vi "test1-testModuleExitEventAPI.vi"(8 "error in (no error)":errorcluster, 11 "TestCase in":refnum<class "testcase-CSMNonCSMCallerSupportAPI.lvclass">) -> (0 "error out":errorcluster, 3 "TestCase out":refnum<class "testcase-CSMNonCSMCallerSupportAPI.lvclass">)   [LabVIEW 2017, in "testcase-CSMNonCSMCallerSupportAPI.lvclass"]
uses:
  testcase-CSMNonCSMCallerSupportAPI.lvclass
  InternalCluster.ctl
  State_Cluster.ctl
  GlobalVariable_CSMModeData.vi
  <vilib>/addons/_JKI Toolkits/VI Tester/TestCase.llb/TestCase.lvclass
  src/user.lib/_NEVSTOP/Communicable State Machine(CSM)/Communicable State Machine.lvlib
  C:/Program Files (x86)/National Instruments/LabVIEW 2017/vi.lib/addons/_JKI Toolkits/VI Tester/TestCase.llb/TestCase.lvclass
panel:
  out "LoopCount":i32
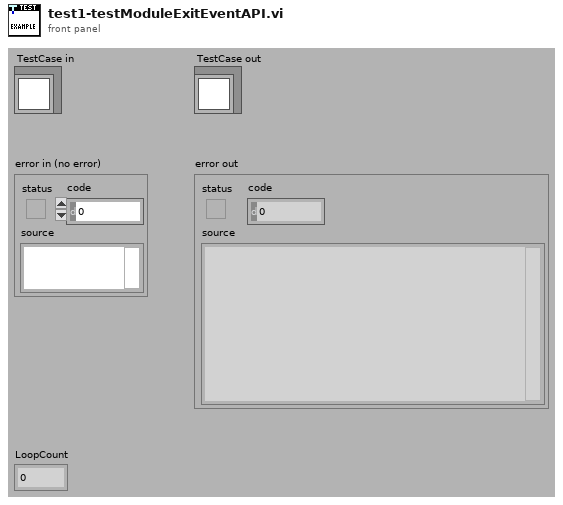
[diagram p1: front panel]
types:
  T1 = typedef "testcase-CSMNonCSMCallerSupportAPI.lvclass/InternalCluster.ctl" = cluster{"Mode":enum16{"Invalid", "Others", "WorkerAgent or Chain"}, "#Nodes":u32}
  T2 = typedef "testcase-CSMNonCSMCallerSupportAPI.lvclass/State_Cluster.ctl" = enum16{"Idle", "Initialize", "PreExit", "Exit"}
  T3 = enum16{"Invalid", "Others", "WorkerAgent or Chain"}
  T4 = typedef "Communicable State Machine.lvlib/_CSM_MODE.ctl" = enum16{"Not Exist", "Stand Alone", "CSM", "Worker", "Worker Agent", "Chain Node", "Chain"}
  T5 = cluster{"Module Exit event occured":bool, "Exit until all nodes exited":bool}
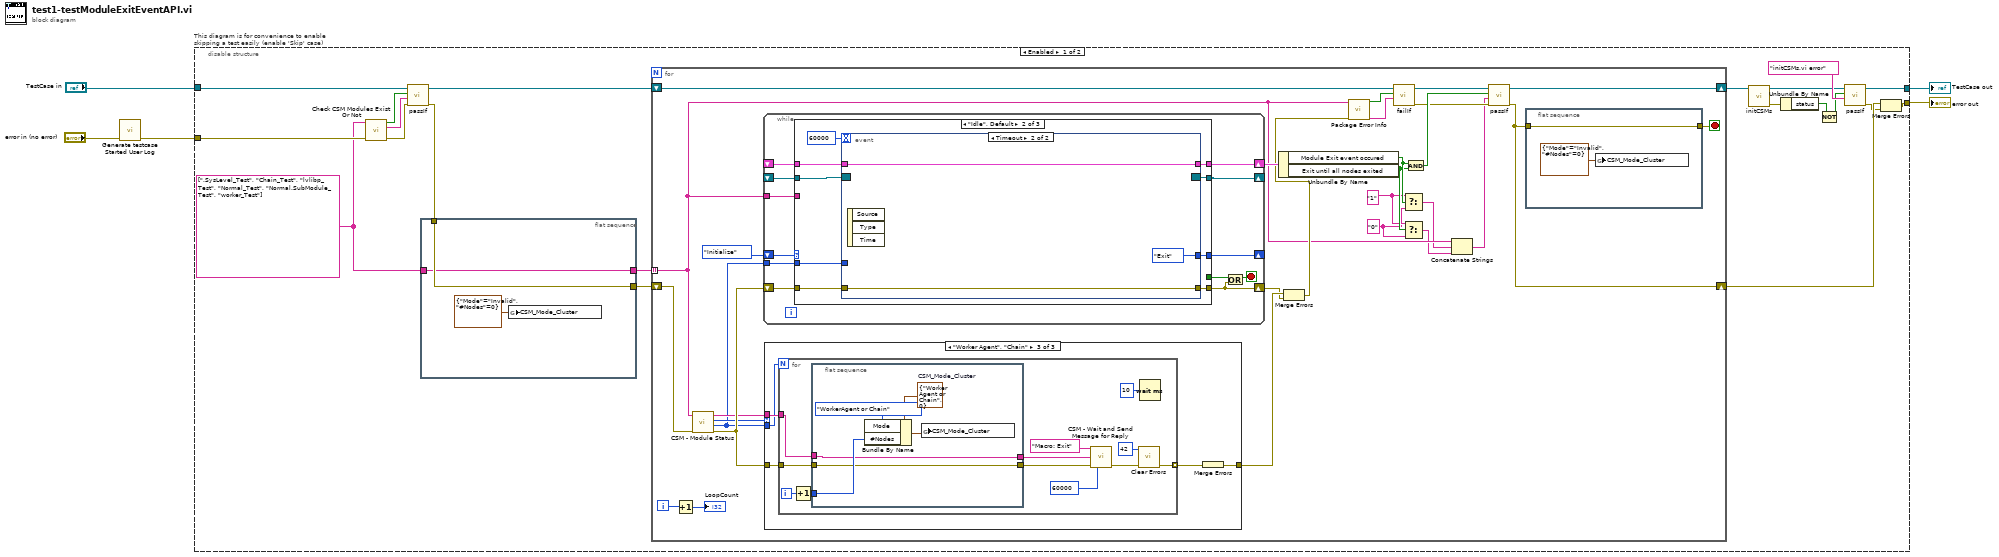
[diagram p0: block diagram]
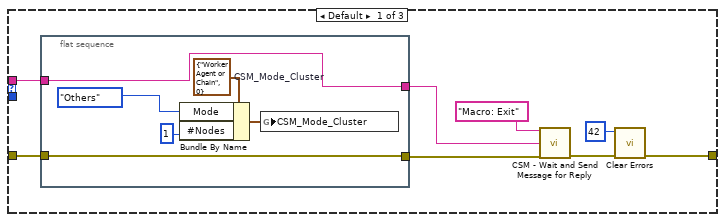
[diagram p2: hidden frame]
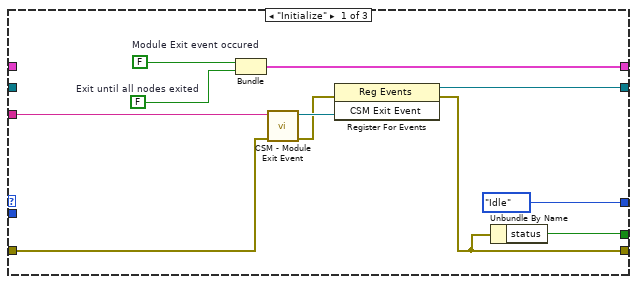
[diagram p4: hidden frame]
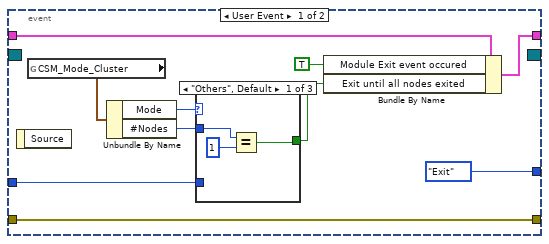
[diagram p5: hidden frame]
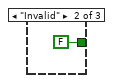
[diagram p6: hidden frame]
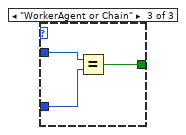
[diagram p7: hidden frame]
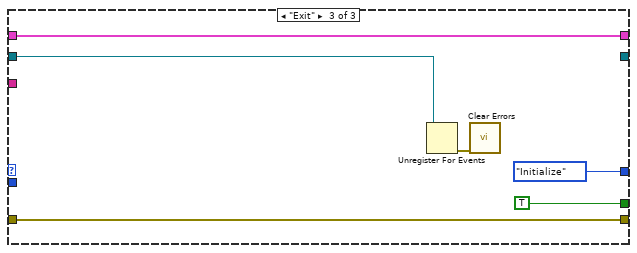
[diagram p8: hidden frame]
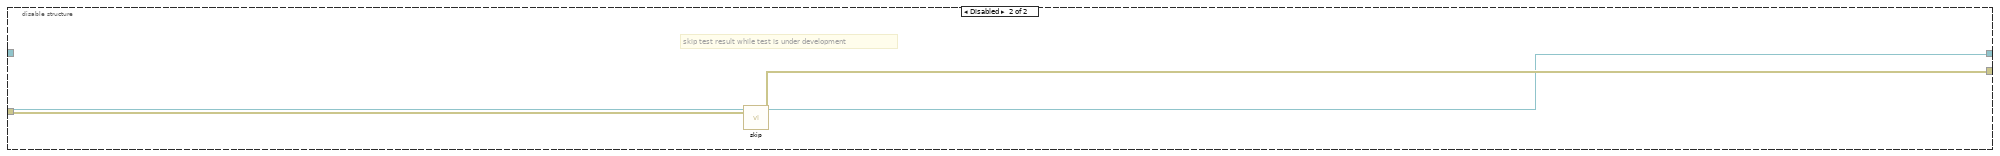
[diagram p9: hidden frame]
diagram:
  n1 = call "Generate testcase Started User Log.vi"("Error In"="error in (no error)") -> ("error out"=w1:errorcluster)  [unwired: 10 in]
  n2 = disable-structure "This diagram is for convenience to enable skipping a test easily (enable 'Skip' case)" shown="Enabled" {
    disable-tunnel: "TestCase in" -> [w18 w159]
    disable-tunnel: [w8 w157] -> w2
    disable-tunnel: [w23 w158] -> w4
    disable-tunnel: w1 -> [w16 w156]
    frame Enabled {
      w6 = string[] [".SysLevel_Test", "Chain_Test", "lvlibp_Test", "Normal_Test", "Normal.SubModule_Test", "worker_Test"] ("Module Names in All Scope")
      n3 = call "Check CSM Modules Exist Or Not.vi"("error in"=w16, "CSM names in"=w6) -> ("error out"=w19:errorcluster, "Debug string"=w20:string, "All Modules Exist?"=w21:bool)  [unwired: 7 in]
      n4 = call-dynamic "passIf.vi"("error in (no error)"=w19, "message (\"\")"=w20, "pass"=w21, "TestCase in"=w18) -> ("error out"=w15:errorcluster, "TestCase out"=w17:refnum<class "testcase-CSMNonCSMCallerSupportAPI.lvclass">)  [unwired: 6 in]
      n5 = flat-sequence {
        tunnel: [w27] -> w25
        tunnel: [w26] -> w22
        tunnel: w15 -> [w27]
        tunnel: w6 -> [w26]
        frame #0 {
          n6 = global write "GlobalVariable_CSMModeData.vi" "CSM_Mode_Cluster"(T1 {"Mode"=enum."Invalid", "#Nodes"=0} ("CSM_Mode_Cluster")) -> ()
        }
      }
      n7 = for {
        shift-right: [w38] -> w14
        shift-left: w25 -> [w52]
        shift-right: [w45] -> w24
        shift-left: w17 -> [w42]
        tunnel: w22 -> [w33] mode=indexing
        i -> [w56]
        stop <- w46 stop-if-true
        w34 = "0"
        w35 = "1"
        n8 = Increment(x=w56) -> (x+1=→"LoopCount":i32)
        n9 = call "CSM - Module Status.vi"("Error In"=w52, "CSM Name"=w33) -> ("error out"=w50:errorcluster, "#Nodes"=w47:i32, "Mode"=w49:T4, "CSM Name (Dup)"=w48:string)  [unwired: 5 in, 1 out]
        n10 = while {
          shift-right: [w105] -> _
          shift-left: State_Cluster."Initialize" -> [w103]
          shift-right: [w108] -> _
          shift-left: _ -> [w107]
          shift-right: [w106] -> w54
          shift-left: _ -> [w104]
          shift-right: [w98] -> w29
          shift-left: w50 -> [w101]
          tunnel: w47 -> [w102]
          tunnel: w33 -> [w100]
          stop <- w99 stop-if-true
          n11 = case shown="\"Idle\", Default" w103 {
            tunnel: [w117 _ TRUE] -> w109
            tunnel: [w119 w128 _] -> w108
            tunnel: w107 -> [_ w129 w155]
            tunnel: [w112 w126 w153] -> w106
            tunnel: w104 -> [_ w127 w153]
            tunnel: w101 -> [w118 w123 w151]
            tunnel: [w115 w122 w151] -> w98
            tunnel: [State_Cluster."Idle" w124 State_Cluster."Initialize"] -> w105
            tunnel: w102 -> [_ w121 _]
            tunnel: w100 -> [w110 _ _]
            frame "Initialize" {
              w111 = FALSE  # Exit until all nodes exited
              w113 = FALSE  # Module Exit event occured
              n12 = Bundle("Module Exit event occured"=w113, "Exit until all nodes exited"=w111) -> (w112:T5)  [unwired: 1 in]
              n13 = call "CSM - Module Exit Event.vi"("Error In"=w118, "Name (\"\" to Use UUID) In"=w110) -> ("error out"=w116:errorcluster, "CSM Exit Event"=w120:refnum<user-event>)  [unwired: 7 in, 1 out]
              n14 = register-events(error in=w116, w120) -> (reference out=w119:refnum<event-registration>, error out=w115:errorcluster)  [unwired: 1 in]
              n15 = Unbundle By Name(w115) -> ("status"=w117:bool)
            }
            frame "Idle", Default {
              n16 = event shown="[1] Timeout" {
                selector: w129 -> [_ _]
                dyn-events: [_ _] -> w128
                timeout: 60000 -> [_ _]
                tunnel: [State_Cluster."Exit" State_Cluster."Exit"] -> w124
                tunnel: w127 -> [w138 w149]
                tunnel: [w131 w149] -> w126
                tunnel: w123 -> [w136 w147]
                tunnel: [w136 w147] -> w122
                tunnel: w121 -> [w132 _]
                event User Event {
                  n17 = event-data() -> ()  [unwired: 1 in, 1 out]
                  n18 = global read "GlobalVariable_CSMModeData.vi" "CSM_Mode_Cluster"() -> (w135:T1)
                  n19 = Unbundle By Name(w135) -> ("Mode"=w134:T3, "#Nodes"=w133:u32)
                  n20 = case shown="\"Others\", Default" w134 {
                    tunnel: [w140 FALSE w144] -> w130
                    tunnel: w133 -> [w142 _ w146]
                    tunnel: w132 -> [_ _ w145]
                    frame "Others", Default {
                      n21 = Equal?(x=w142, y=u32 1) -> (x = y?=w140:bool)
                    }
                    frame "Invalid" {
                    }
                    frame "WorkerAgent or Chain" {
                      n22 = Equal?(x=w146, y=w145) -> (x = y?=w144:bool)
                    }
                  }
                  n23 = Bundle By Name(cluster=w138, "Module Exit event occured"=TRUE, "Exit until all nodes exited"=w130) -> (w131:T5)
                }
                event Timeout {
                  n24 = event-data() -> ()  [unwired: 1 in, 3 out]
                }
              }
            }
            frame "Exit" {
              n25 = Unregister For Events(event registration refnum=w155) -> (error out=w154:errorcluster)  [unwired: 1 in]
              n26 = call <vilib>:"Clear Errors.vi"("error in (no error)"=w154) -> ()  [unwired: 5 in, 2 out]
            }
          }
          n27 = Or(x=w109, y=w98) -> (x .or. y?=w99:bool)
        }
        n28 = case shown="\"Worker Agent\", \"Chain\"" w49 {
          tunnel: w50 -> [w61 w74 w79]
          tunnel: w47 -> [_ _ w77]
          tunnel: w48 -> [w63 _ w78]
          tunnel: [w65 w74 w75] -> w51
          frame Default {
            n29 = flat-sequence {
              tunnel: w63 -> [w69]
              tunnel: [w69] -> w62
              tunnel: w61 -> [w68]
              tunnel: [w68] -> w60
              frame #0 {
                w73 = T1 {"Mode"=enum."WorkerAgent or Chain", "#Nodes"=0}  # CSM_Mode_Cluster
                n30 = Bundle By Name(cluster=w73, "Mode"=T3."Others", "#Nodes"=u32 1) -> (w72:T1)
                n31 = global write "GlobalVariable_CSMModeData.vi" "CSM_Mode_Cluster"(w72) -> ()
              }
            }
            n32 = call "CSM - Wait and Send Message for Reply.vi"("State"="Macro: Exit", "Target Module"=w62, "Error In (No Error)"=w60) -> ("error out"=w66:errorcluster)  [unwired: 9 in, 3 out]
            n33 = call <vilib>:"Clear Errors.vi"("error in (no error)"=w66, "specific error code to clear (0: all)"=42) -> ("error out"=w65:errorcluster)  [unwired: 4 in, 1 out]
          }
          frame "Not Exist" {
          }
          frame "Worker Agent", "Chain" {
            n34 = for {
              N: w77 -> [_]
              tunnel: w78 -> [w84]
              tunnel: w79 -> [w82]
              tunnel: [w87] -> w76 mode=indexing
              i -> [w90]
              n35 = Increment(x=w90) -> (x+1=w89:i32)
              n36 = flat-sequence {
                tunnel: w89 -> [w95]
                tunnel: w84 -> [w93]
                tunnel: [w93] -> w83
                tunnel: w82 -> [w92]
                tunnel: [w92] -> w81
                frame #0 {
                  w97 = T1 {"Mode"=enum."WorkerAgent or Chain", "#Nodes"=0}  # CSM_Mode_Cluster
                  n37 = Bundle By Name(cluster=w97, "Mode"=T3."WorkerAgent or Chain", "#Nodes"=w95) -> (w96:T1)
                  n38 = global write "GlobalVariable_CSMModeData.vi" "CSM_Mode_Cluster"(w96) -> ()
                }
              }
              n39 = call "CSM - Wait and Send Message for Reply.vi"("State"="Macro: Exit", "Target Module"=w83, "Error In (No Error)"=w81, "Response Timeout (-2 Using Global Settings)"=60000) -> ("error out"=w88:errorcluster)  [unwired: 8 in, 3 out]
              n40 = call <vilib>:"Clear Errors.vi"("error in (no error)"=w88, "specific error code to clear (0: all)"=42) -> ("error out"=w87:errorcluster)  [unwired: 4 in, 1 out]
              n41 = Wait (ms)(milliseconds to wait=u32 10) -> ()  [unwired: 1 out]
            }
            n42 = Merge Errors(w76) -> (w75:errorcluster)
          }
        }
        n43 = Unbundle By Name(w54) -> ("Module Exit event occured"=w37:bool, "Exit until all nodes exited"=w36:bool)
        n44 = Merge Errors(w51, w29) -> (w39:errorcluster)
        n45 = call "Package Error Info.vi"("error in"=w39, "String in"=w33) -> ("packed error info out"=w43:string, "error status"=w44:bool)  [unwired: 8 in]
        n46 = call-dynamic "failIf.vi"("message (\"\")"=w43, "fail"=w44, "TestCase in"=w42) -> ("error out"=w40:errorcluster, "TestCase out"=w41:refnum<class "testcase-CSMNonCSMCallerSupportAPI.lvclass">)  [unwired: 7 in]
        n47 = Select(t=w35, s=w37, f=w34) -> (s? t:f=w32:string)
        n48 = Select(t=w35, s=w36, f=w34) -> (s? t:f=w31:string)
        n49 = And(x=w37, y=w36) -> (x .and. y?=w53:bool)
        n50 = Concatenate Strings(w33, w32, w31) -> (w30:string)
        n51 = call-dynamic "passIf.vi"("error in (no error)"=w40, "message (\"\")"=w30, "pass"=w53, "TestCase in"=w41) -> ("error out"=w38:errorcluster, "TestCase out"=w45:refnum<class "testcase-CSMNonCSMCallerSupportAPI.lvclass">)  [unwired: 6 in]
        n52 = flat-sequence {
          tunnel: w38 -> [w58]
          tunnel: [w58] -> w46
          frame #0 {
            n53 = global write "GlobalVariable_CSMModeData.vi" "CSM_Mode_Cluster"(T1 {"Mode"=enum."Invalid", "#Nodes"=0} ("CSM_Mode_Cluster")) -> ()
          }
        }
      }
      n54 = call "initCSMs.vi"("TestCase in"=w24) -> ("error out"=w10:errorcluster, "TestCase out"=w9:refnum<class "testcase-CSMNonCSMCallerSupportAPI.lvclass">)  [unwired: 9 in]
      n55 = Unbundle By Name(w10) -> ("status"=w11:bool)
      n56 = Not(x=w11) -> (.not. x?=w12:bool)
      n57 = call-dynamic "passIf.vi"("message (\"\")"="initCSMs.vi error" ("message (\"\")"), "pass"=w12, "TestCase in"=w9) -> ("error out"=w7:errorcluster, "TestCase out"=w8:refnum<class "testcase-CSMNonCSMCallerSupportAPI.lvclass">)  [unwired: 7 in]
      n58 = Merge Errors(w14, w7) -> (w23:errorcluster)
    }
    frame Disabled {
      # "skip test result while test is under development"
      n59 = call <vilib>:"skip.vi"("error in (no error)"=w156, "TestCase in"=w159) -> ("error out"=w158:errorcluster, "TestCase out"=w157:refnum<class "testcase-CSMNonCSMCallerSupportAPI.lvclass">)  [unwired: 8 in]
    }
  }
  "error out" <- w4
  "TestCase out" <- w2
